vi "New Channel.vi"(8 "error in (no error)":errorcluster, 11 "ChannelManagerUI in":refnum<class "ChannelManagerUI.lvclass">) -> (0 "error out":errorcluster, 3 "ChannelManagerUI out":refnum<class "ChannelManagerUI.lvclass">)   [LabVIEW 2021, in "Channel.lvlib" / "ChannelManagerUI.lvlib" / "ChannelManagerUI.lvclass"]
uses:
  ChannelManagerUI.lvclass
  ChannelManagerUI.lvclass/ChannelManagerUI.ctl
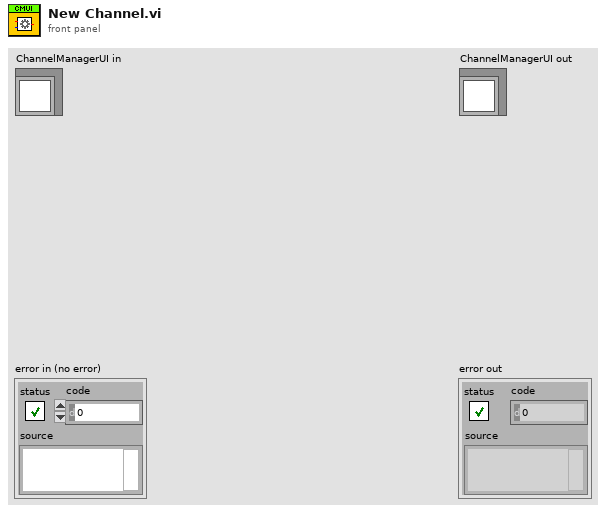
[diagram p1: front panel]
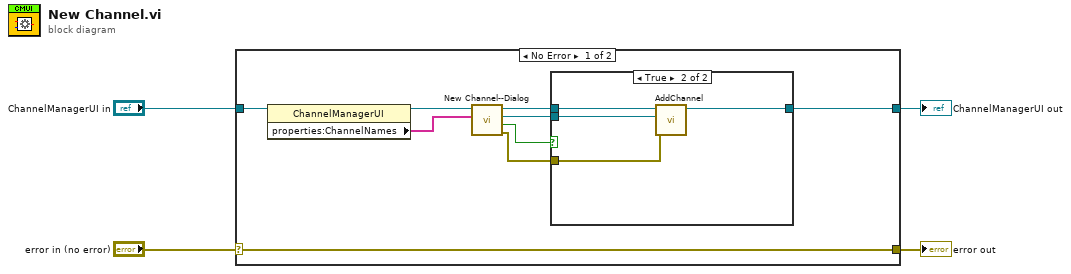
[diagram p0: block diagram]
diagram:
  n1 = case shown="No Error" "error in (no error)" {
    selector: "error in (no error)" -> [w12 w20]
    tunnel: [w12 w20] -> w3
    tunnel: [w9 w19] -> w1
    tunnel: "ChannelManagerUI in" -> [w13 w19]
    frame No Error {
      n2 = property class="ChannelManagerUI"(reference=w13) -> (reference out=w11:refnum<class "ChannelManagerUI.lvclass">, "properties:ChannelNames"=w10:string[])  [unwired: 1 in, 1 out]
      n3 = call-dynamic "New Channel--Dialog.vi"("Channels"=w10, "ChannelManagerUI in"=w11) -> ("error out"=w5:errorcluster, "OK"=w7:bool, "Class"=w6:refnum<class "Channel.lvclass">, "ChannelManagerUI out"=w8:refnum<class "ChannelManagerUI.lvclass">)  [unwired: 6 in]
      n4 = case shown="True" w7 {
        tunnel: [w14 w17] -> w9
        tunnel: w8 -> [w14 w18]
        tunnel: w6 -> [_ w16]
        tunnel: w5 -> [_ w15]
        frame False {
        }
        frame True {
          n5 = call-dynamic "AddChannel.vi"("error in (no error)"=w15, "Channel"=w16, "object in"=w18) -> ("object out"=w17:refnum<class "ChannelManagerUI.lvclass">)  [unwired: 7 in, 1 out]
        }
      }
    }
    frame Error {
    }
  }
  "error out" <- w3
  "ChannelManagerUI out" <- w1
